vi "Dispatch Probe 3.vi"() -> (0 "answer":string)   [LabVIEW 2026]
doc: "Round15 P15 v3: the static-launderer chain. seed (class constant) feeds Sensor:Carrier, a STATIC member, whose obj out is a Sensor-typed wire; that wire feeds the dynamic call Sensor:Tag. The editor cannot bind Tag at edit time (the wire is parent-typed), so the runtime value must select the implementation. answer=Temp Sensor while callTargets still name Sensor members is the proof of dynamic dispatch."
uses:
  lib/Temp Sensor.lvclass
  C:/Users/heiyashi/WorkBuddy/automation-2026-10-18-03-19-34/labview-vi-mcp/research/artifacts/round15/p15/lib/Sensor.lvclass
  lib/Sensor.lvclass
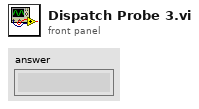
[diagram p1: front panel]
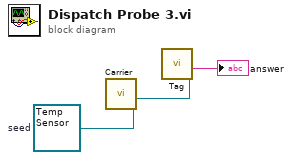
[diagram p0: block diagram]
diagram:
  w1 = refnum<class "Temp Sensor.lvclass"> refnum  # seed
  n1 = call "Carrier.vi"("obj in"=w1) -> ("obj out"=w3:refnum<class "Temp Sensor.lvclass">)  [unwired: 10 in]
  n2 = call-dynamic "Tag.vi"("obj in"=w3) -> ("tag"=→"answer":string)  [unwired: 10 in]
